vi "MS_IDX formation.vi"(8 "AS_ISX":i32, 11 "Sample sequnce":string="CAGACTTTTATTTCTCGCCATAATTCAAACTTTTTTTCTGATAAGCTGGTTCTCACTTCTGTTACTCCAGCTTCTTCGGCACCTGTTTTACAGACACCTAAAGCTACATCGTCAACGTTA") -> (0 "element":string, 2 "MS_IXD3":i32, 3 "MS_IXD5":i32)   [LabVIEW 2018]
panel:
  out "element 2":string
  out "Array 5":i32[](array[numeric])
  out "Array 4":string[](array[string])
  out "size(s)":i32
  out "Array 3":i32[](array[numeric])
  out "Array 2":string[](array[string])
  out "Array":string[](array[string])
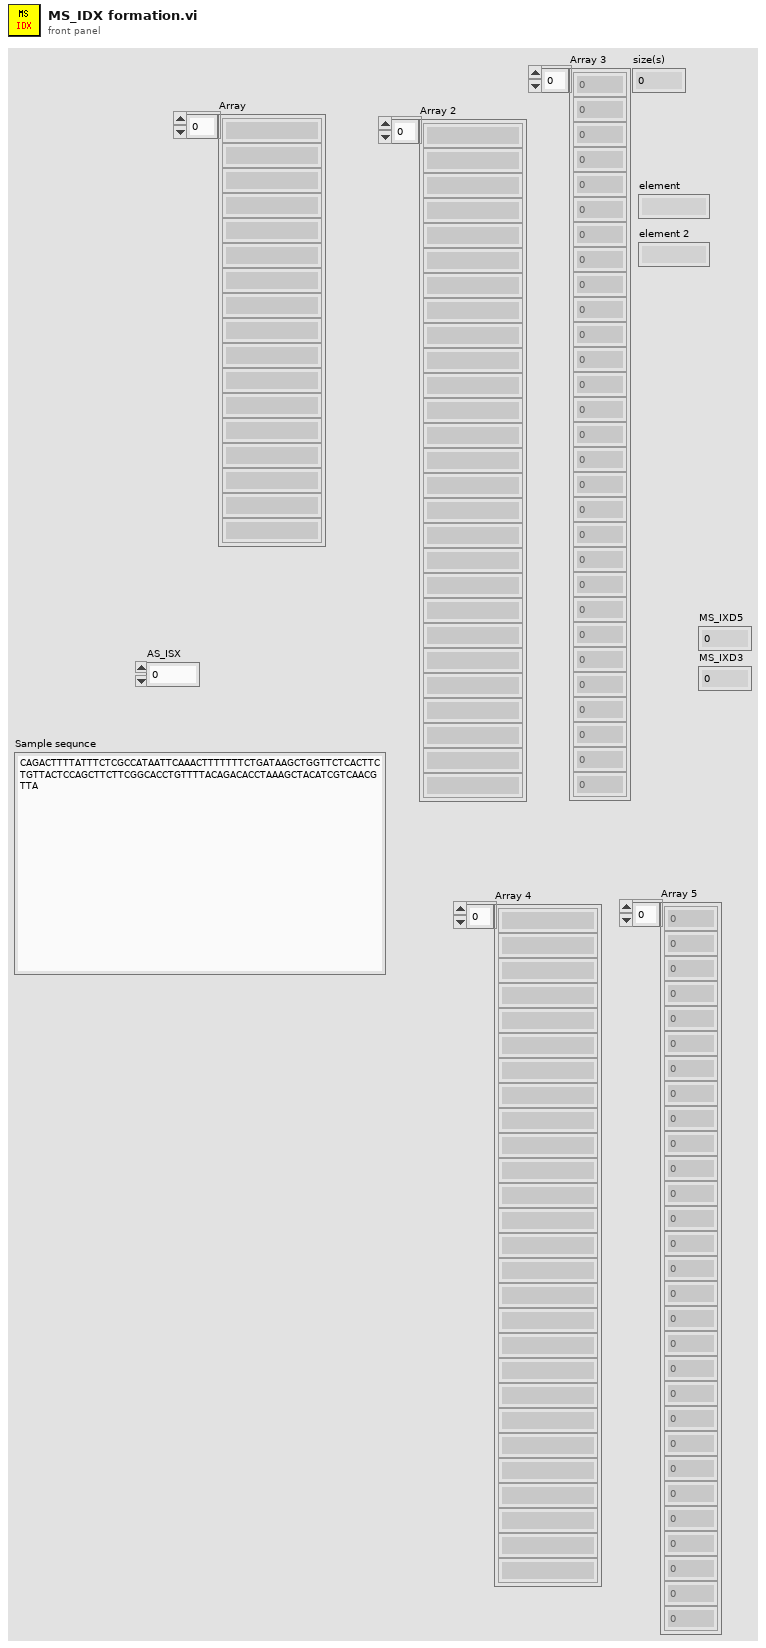
[diagram p1: front panel]
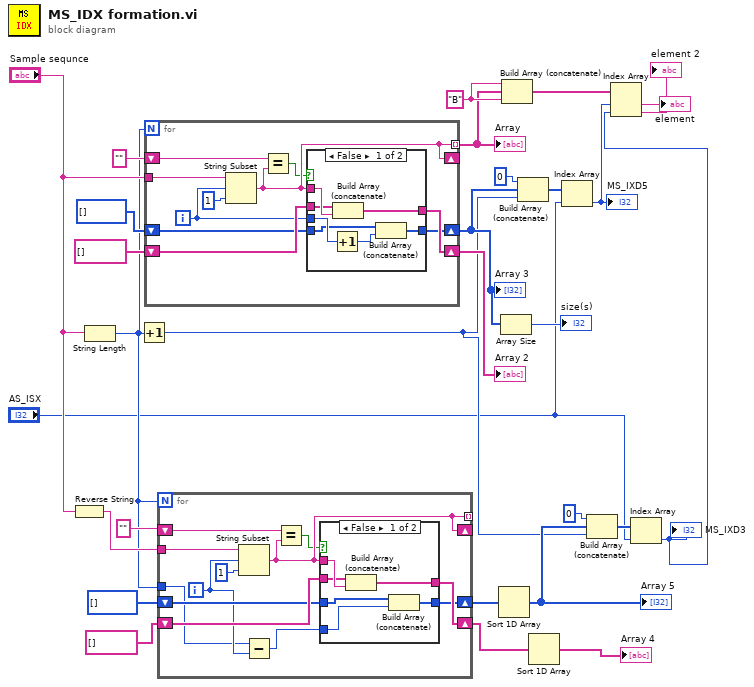
[diagram p0: block diagram]
diagram:
  w21 = "B"
  n1 = Reverse String(1:"Sample sequnce") -> (0:w16:string)
  n2 = String Length(string="Sample sequnce") -> (length=w12:i32)
  n3 = Increment(x=w12) -> (x+1=w4:i32)
  n4 = for {
    N: w12 -> [_]
    tunnel: "Sample sequnce" -> [w39]
    tunnel: [w36] -> w20 mode=indexing
    shift-right: [w36] -> _
    shift-left: "" -> [w37]
    shift-right: [w34] -> w26
    shift-left: string[] [] -> [w33]
    shift-right: [w31] -> w8
    shift-left: i32[] [] -> [w30]
    i -> [w32]
    n5 = String Subset(string=w39, offset (0)=w32, length (rest)=1 ("length (rest)")) -> (substring=w36:string)
    n6 = Equal?(x=w37, y=w36) -> (x = y?=w35:bool)
    n7 = case shown="False" w35 {
      tunnel: w36 -> [w46 _]
      tunnel: [w45 w48] -> w34
      tunnel: w33 -> [w44 w48]
      tunnel: w32 -> [w43 _]
      tunnel: [w42 w47] -> w31
      tunnel: w30 -> [w41 w47]
      frame False {
        n8 = Increment(x=w43) -> (x+1=w40:i32)
        n9 = Build Array (concatenate)(w44, w46) -> (w45:string[])
        n10 = Build Array (concatenate)(w41, w40) -> (w42:i32[])
      }
      frame True {
      }
    }
  }
  "Array" <- w20
  "Array 2" <- w26
  "Array 3" <- w8
  n11 = for {
    N: w12 -> [_]
    tunnel: w16 -> [w60]
    tunnel: [w57] -> _ mode=indexing
    shift-right: [w57] -> _
    shift-left: "" -> [w58]
    shift-right: [w55] -> w10
    shift-left: string[] [] -> [w54]
    shift-right: [w53] -> w11
    shift-left: i32[] [] -> [w52]
    tunnel: w12 -> [w50]
    i -> [w51]
    n12 = String Subset(string=w60, offset (0)=w51, length (rest)=1 ("length (rest)")) -> (substring=w57:string)
    n13 = Subtract(x=w50, y=w51) -> (x-y=w49:i32)
    n14 = Equal?(x=w58, y=w57) -> (x = y?=w56:bool)
    n15 = case shown="False" w56 {
      tunnel: w57 -> [w66 _]
      tunnel: [w65 w68] -> w55
      tunnel: w54 -> [w64 w68]
      tunnel: [w63 w67] -> w53
      tunnel: w52 -> [w62 w67]
      tunnel: w49 -> [w61 _]
      frame False {
        n16 = Build Array (concatenate)(w64, w66) -> (w65:string[])
        n17 = Build Array (concatenate)(w62, w61) -> (w63:i32[])
      }
      frame True {
      }
    }
  }
  n18 = Sort 1D Array(array=w11) -> (sorted array=w5:i32[])
  "Array 5" <- w5
  n19 = Array Size(array=w8) -> (size(s)=→"size(s)":i32)
  n20 = Build Array (concatenate)(w21, w20, w21) -> (w19:string[])
  n21 = Build Array (concatenate)(0 ("length (rest)"), w8, w4) -> (w23:i32[])
  n22 = Sort 1D Array(array=w10) -> (sorted array=→"Array 4":string[])
  n23 = Index Array(array=w23, index="AS_ISX") -> (element=w18:i32)
  "MS_IXD5" <- w18
  n24 = Build Array (concatenate)(0 ("length (rest)"), w5, w4) -> (w6:i32[])
  n25 = Index Array(array=w6, index="AS_ISX") -> (element=w2:i32)
  "MS_IXD3" <- w2
  n26 = Index Array(array=w19, index #1=w18, index #2=w2) -> (element #1=→"element":string, element #2=→"element 2":string)
